vi "Callback Change Channel Name.vi"(6 "Variant":variant, 8 "error in (no error)":errorcluster, 9 "Old Values":string[][](array[string]), 10 "object ref in":T1, 11 "Table Change":T2) -> (0 "error out":errorcluster)   [LabVIEW 2015, in "DAQmx Module editor node.lvclass"]
doc: "This VI gets called automatically when changes are made to the 'Name' column of the table and must handle changes appropriately. Register this callback using the appropriate 'Define Column' VI from the Table API."
uses:
  DAQmx Module editor node.lvclass
  <vilib>/NI/DCAF/Tag Editor Core/Table API/Table Manager/Cell Change.ctl
  <vilib>/NI/DCAF/Tag Editor Core/Table API/Table Manager/object ref.ctl
  <vilib>/NI/DCAF/Tag Editor Core/Configuration Editor/Classes/Engine Parent/Engine Parent Editor Node.lvclass
  <vilib>/NI/DCAF/Tag Editor Core/Configuration Editor/Classes/Module editor node/module editor node.lvclass
  module/configuration/Daqmx Module configuration.lvclass
  module/configuration/Daqmx Module configuration.lvclass/Daqmx Module configuration.ctl
  <vilib>/NI/Configuration Framework/serializable configuration/NISE_CEF_serializable configuration.lvclass/NISE_CEF_serializable configuration.ctl
  <vilib>/NI/Tag Bus/tag/tag descriptor.lvclass/tag descriptor.ctl
  <vilib>/Utility/LVClass/Get LV Class Name.vi
  <vilib>/NI/Configuration Framework/error generator/NISE_error generator.vi
  module/configuration/Get Line Name.vi
  <vilib>/NI/Tag Bus Module Framework/module configuration/FindDuplicate.vi
  <vilib>/Utility/error.llb/Error Cluster From Error Code.vi
  <vilib>/NI/Tag Bus Module Framework/channel/TBM channel.lvclass
  <vilib>/NI/Module Execution Interface/Engine Configuration/engine configuration.lvclass
  <vilib>/NI/Tag Bus/tag/tag descriptor.lvclass
  <vilib>/NI/Configuration Framework/serializable configuration/NISE_CEF_serializable configuration.lvclass
  <vilib>/NI/DCAF/Tag Editor Core/Table API/Table Manager.lvlib
  <vilib>/NI/DCAF/Tag Editor Core/Table API/Table Manager/Table Manager.lvclass
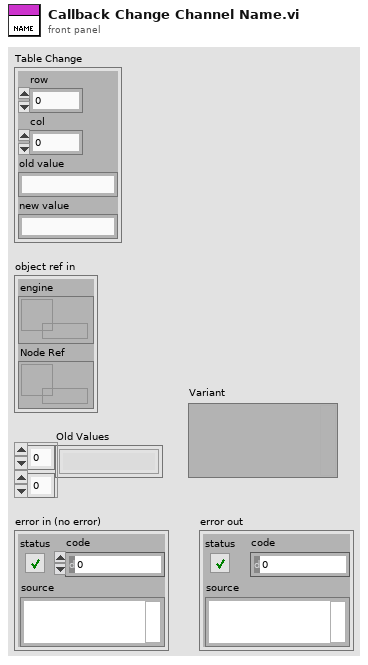
[diagram p1: front panel]
types:
  T1 = typedef "Table Manager.lvlib/Table Manager.lvclass/object ref.ctl" = cluster{"engine":refnum<data-value>, "Node Ref":refnum<data-value>}
  T2 = typedef "Table Manager.lvlib/Cell Change.ctl" = cluster{"row":i32, "col":i32, "old value":string, "new value":string}
  T3 = typedef "DAQmx Module Configuration.lvclass/Line.ctl" = cluster{"Channel Array":refnum<class "TBM channel.lvclass">[], "Physical Channel":string, "Measurement Type":T4, "Parameters":T5}
  T4 = typedef "DAQmx Module Configuration.lvclass/Measurement Type.ctl" = enum16{"Digital Input", "Digital Output", "Voltage Input", "Voltage Output", "Current Input", "Current Output", "RTD", "Thermocouple", "Strain", "PWM"}
  T5 = typedef "DAQmx Module Configuration.lvclass/Parameters.ctl" = cluster{"Digital Config":cluster{"Invert Lines?":bool}, "Voltage Config":cluster{"Maximum Value (V)":dbl, "Minimum Value (V)":dbl, "in terminal configuration (V)":i32, "out terminal configuration (V)":i32}, "Current Config":cluster{"Maximum Value (A)":dbl, "Minimum Value (A)":dbl, "shunt resistor location":i32, "input terminal configuration (C)":i32, "external shunt resistor value":dbl}, "RTD Config":cluster{"Maximum Value (°C)":dbl, "Minimum Value (°C)":dbl, "resistance configuration":i32, "r0":dbl, "current excitation value":dbl, "rtd type":i32, "current excitation source":i32}, "Thermocouple Config":cluster{"Minimum Value (C)":dbl, "Maximum Value (C)":dbl, "thermocouple type":i32, "cjc source":i32, "cjc value":dbl}, "Strain Config":cluster{"Maximum Value":dbl, "Minimum Value":dbl, "bridge information":cluster{"strain configuration":i32, "lead wire resistance":dbl, "initial bridge voltage":dbl, "voltage excitation source":i32, "voltage excitation value":dbl}, "strain gage information":cluster{"gage factor":dbl, "nominal gage resistance":dbl, "poisson ratio":dbl}}, "PWM Config":cluster{"Idle State":bool}}
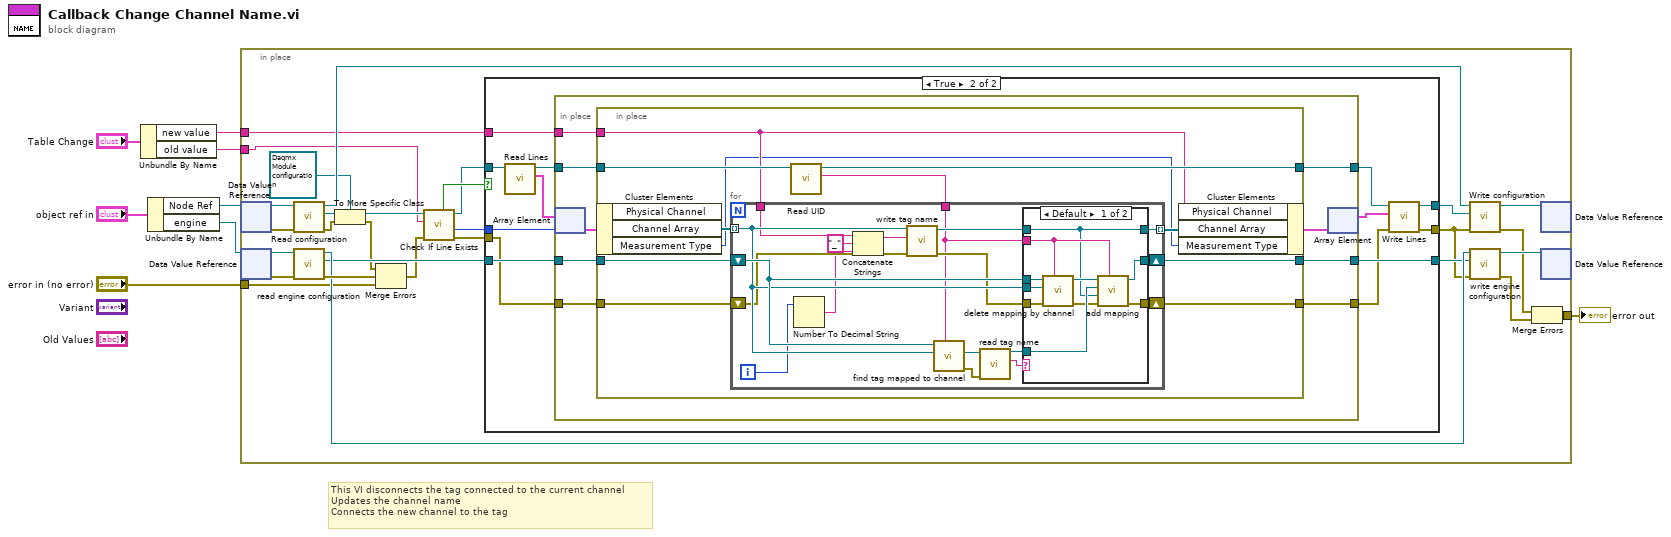
[diagram p0: block diagram]
diagram:
  # "This VI disconnects the tag connected to the current channel\nUpdates the channel name\nConnects the new channel to the tag"
  n1 = Unbundle By Name("Table Change") -> ("new value"=w1:string, "old value"=w2:string)
  n2 = Unbundle By Name("object ref in") -> ("Node Ref"=w5:refnum<data-value>, "engine"=w4:refnum<data-value>)
  n3 = in-place {
    in-place-border: [w29] -> w8
    in-place-border: "error in (no error)" -> [w25]
    in-place-border: w2 -> [w9]
    in-place-border: w1 -> [w21]
    n4 = in-place-dvr #1(w5) -> (w19:refnum<class "module editor node.lvclass">, w28:errorcluster)
    n5 = in-place-dvr #2(w4) -> (w36:refnum<class "Engine Parent Editor Node.lvclass">, w37:errorcluster)
    n6 = call-dynamic "Read configuration.vi"("error in"=w28, "NISE_CEF_serializable node in"=w19) -> ("error out"=w11:errorcluster, "configuration"=w26:refnum<class "NISE_CEF_serializable configuration.lvclass">, "NISE_CEF_serializable node out"=w27:refnum<class "module editor node.lvclass">)  [unwired: 7 in]
    n7 = call <vilib>:"read engine configuration.vi"("error in"=w37, "Engine Parent Editor Node in"=w36) -> ("error out"=w33:errorcluster, "engine configuration"=w16:refnum<class "engine configuration.lvclass">, "Engine Parent Editor Node out"=w32:refnum<class "Engine Parent Editor Node.lvclass">)  [unwired: 7 in]
    n8 = To More Specific Class(target class=refnum<class "Daqmx Module configuration.lvclass"> refnum ("tag bus configurable plugin module configuration"), reference=w26, error in=w11) -> (specific class reference=w18:refnum<class "Daqmx Module configuration.lvclass">, error out=w10:errorcluster)
    n9 = Merge Errors(w10, w33, w25) -> (w14:errorcluster)
    n10 = call-dynamic "Check If Line Exists.vi"("error in"=w14, "Name to Locate"=w9, "Daqmx Module configuration in"=w18) -> ("error out"=w15:errorcluster, "Index"=w22:i32, "Daqmx Module configuration out"=w13:refnum<class "Daqmx Module configuration.lvclass">, "Found?"=w20:bool)  [unwired: 4 in, 1 out]
    n11 = case shown="True" w20 {
      tunnel: [w40 w53] -> w23
      tunnel: w13 -> [w40 w52]
      tunnel: w22 -> [_ w49]
      tunnel: w21 -> [_ w48]
      tunnel: w16 -> [w39 w47]
      tunnel: [w39 w46] -> w17
      tunnel: [w38 w45] -> w12
      tunnel: w15 -> [w38 w43]
      frame False {
      }
      frame True {
        n12 = call "Read Lines.vi"("Daqmx Module configuration in"=w52) -> ("Lines"=w51:T3[], "Daqmx Module configuration out"=w42:refnum<class "Daqmx Module configuration.lvclass">)  [unwired: 8 in, 1 out]
        n13 = in-place {
          in-place-border: w48 -> [w60]
          in-place-border: w47 -> [w59]
          in-place-border: [w58] -> w46
          in-place-border: [w57] -> w44
          in-place-border: w43 -> [w56]
          in-place-border: w42 -> [w55]
          in-place-border: [w54] -> w41
          n14 = in-place-array #3(w51, w49) -> (w62:T3)
          n15 = in-place {
            in-place-border: w60 -> [w64]
            in-place-border: w59 -> [w72]
            in-place-border: [w73] -> w58
            in-place-border: [w69] -> w57
            in-place-border: w56 -> [w70]
            in-place-border: w55 -> [w67]
            in-place-border: [w66] -> w54
            n16 = in-place-cluster #4(w62) -> ("Channel Array"=w71:refnum<class "TBM channel.lvclass">[], "Measurement Type"=w63:T4)  [unwired: 1 out]
            n17 = call <vilib>:"Read UID.vi"("configuration in"=w67) -> ("instance id"=w68:string, "configuration out"=w66:refnum<class "Daqmx Module configuration.lvclass">)  [unwired: 8 in, 1 out]
            n18 = for {
              tunnel: w71 -> [w89] mode=indexing
              tunnel: w68 -> [w81]
              tunnel: [w80] -> w65 mode=indexing
              tunnel: w64 -> [w78]
              shift-right: [w91] -> w73
              shift-left: w72 -> [w90]
              shift-right: [w82] -> w69
              shift-left: w70 -> [w84]
              i -> [w76]
              n19 = Number To Decimal String(number=w76) -> (decimal integer string=w75:string)  [unwired: 1 in]
              n20 = Concatenate Strings(w78, "_" ("string"), w75) -> (w77:string)
              n21 = call <vilib>:"write tag name.vi"("error in"=w84, "name"=w77, "system tag in"=w89) -> ("error out"=w83:errorcluster, "system tag out"=w85:refnum<class "TBM channel.lvclass">)  [unwired: 7 in]
              n22 = call <vilib>:"find tag mapped to channel.vi"("owner"=w81, "channel"=w89, "engine configuration in"=w90) -> ("error out"=w79:errorcluster, "tag"=w88:refnum<class "tag descriptor.lvclass">)  [unwired: 6 in, 1 out]
              n23 = call <vilib>:"read tag name.vi"("error in"=w79, "system tag in"=w88) -> ("name"=w87:string, "system tag out"=w86:refnum<class "tag descriptor.lvclass">)  [unwired: 7 in, 1 out]
              n24 = case shown="Default" w87 {
                tunnel: [w100 w104] -> w91
                tunnel: w90 -> [w99 w104]
                tunnel: w81 -> [w98 _]
                tunnel: w89 -> [w97 _]
                tunnel: w86 -> [w96 _]
                tunnel: w85 -> [w92 w102]
                tunnel: [w94 w103] -> w82
                tunnel: w83 -> [w93 w103]
                tunnel: [w92 w102] -> w80
                frame Default {
                  n25 = call <vilib>:"delete mapping by channel.vi"("owner ID"=w98, "error in"=w93, "channel"=w97, "engine configuration in"=w99) -> ("error out"=w95:errorcluster, "engine configuration out"=w101:refnum<class "engine configuration.lvclass">)  [unwired: 6 in]
                  n26 = call-dynamic "add mapping.vi"("owner ID"=w98, "error in"=w95, "channel"=w92, "tag descriptor"=w96, "engine configuration"=w101) -> ("error out"=w94:errorcluster, "engine configuration out"=w100:refnum<class "engine configuration.lvclass">)  [unwired: 5 in]
                }
                frame "" {
                }
              }
            }
            n27 = in-place-cluster #4("Physical Channel"=w64, "Channel Array"=w65, "Measurement Type"=w63) -> (w61:T3)
          }
          n28 = in-place-array #3(w61) -> (w50:T3[])  [unwired: 1 out]
        }
        n29 = call "Write Lines.vi"("error in (no error)"=w44, "Lines"=w50, "Daqmx Module configuration in"=w41) -> ("error out"=w45:errorcluster, "Daqmx Module configuration out"=w53:refnum<class "Daqmx Module configuration.lvclass">)  [unwired: 7 in]
      }
    }
    n30 = call-dynamic "Write configuration.vi"("error in"=w12, "configuration"=w23, "NISE_CEF_serializable node in"=w27) -> ("error out"=w30:errorcluster, "NISE_CEF_serializable node out"=w34:refnum<class "module editor node.lvclass">)  [unwired: 7 in]
    n31 = call <vilib>:"write engine configuration.vi"("error in"=w12, "engine configuration"=w17, "Engine Parent Editor Node in"=w32) -> ("error out"=w31:errorcluster, "Engine Parent Editor Node out"=w35:refnum<class "Engine Parent Editor Node.lvclass">)  [unwired: 7 in]
    n32 = Merge Errors(w30, w31) -> (w29:errorcluster)
    n33 = in-place-dvr #1(w34) -> ()  [unwired: 2 out]
    n34 = in-place-dvr #2(w35) -> ()  [unwired: 2 out]
  }
  "error out" <- w8
